vi "Offset Measurement Next Phase.vi"(6 "zero":T1, 8 "error in (no error)":errorcluster, 9 "Status":T4=enum."created", 10 "Offset Measurement":T2={"phase"=enum."idle", "measureInputOffset"={"buffers"=0, "settle"=2, "timeout"=5.0, "channels"=[], "zero"=enum."both"}, "settle remaining"=0, "buffers remaining"=0, "deadline"=0, "sum"=[], "count"=0, "saved amplitudes"=[], "saved offsets"=[], "previous status"=enum."created"}, 11 "Instrument.DAQ in":refnum<class "Instrument.DAQ.lvclass">) -> (0 "error out":errorcluster, 2 "Offset Measurement":T2={"phase"=enum."idle", "measureInputOffset"={"buffers"=0, "settle"=2, "timeout"=5.0, "channels"=[], "zero"=enum."both"}, "settle remaining"=0, "buffers remaining"=0, "deadline"=0, "sum"=[], "count"=0, "saved amplitudes"=[], "saved offsets"=[], "previous status"=enum."created"}, 3 "Instrument.DAQ out":refnum<class "Instrument.DAQ.lvclass">)   [LabVIEW 2019, in "Instrument.Lockin.lvlib" / "Instrument.DAQ.lvclass"]
uses:
  Instrument.DAQ.lvclass
  Typedefs/Offset Measurement--Cluster.ctl
  Lockin.Typedefs/API/Lockin.measureInputOffset Config--Cluster.ctl
  Lockin.Typedefs/API/Lockin.measureInputOffset.zero--enum.ctl
  Lockin.Typedefs/other/Status--enum.ctl
  Instrument.DAQ.lvclass/Instrument.DAQ.ctl
  Lockin.Typedefs/Lockin.Typedefs.lvlib
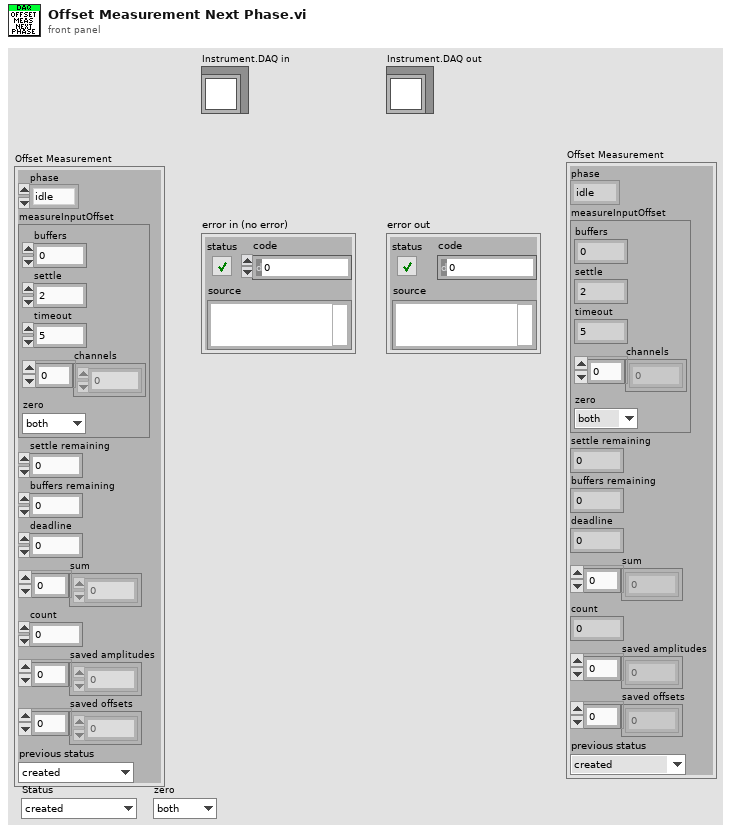
[diagram p1: front panel]
types:
  T1 = typedef "Lockin.Typedefs.lvlib/Lockin.measureInputOffset.zero--enum.ctl" = enum16{"both", "ac", "dc", "none"}
  T2 = typedef "Instrument.Lockin.lvlib/Instrument.DAQ.lvclass/Offset Measurement--Cluster.ctl" = cluster{"phase":enum16{"idle", "zeroing", "settling", "averaging", "done", "aborted", "cancelled", "timed out"}, "measureInputOffset":T3, "settle remaining":i32, "buffers remaining":i32, "deadline":u32, "sum":dbl[], "count":i32, "saved amplitudes":dbl[], "saved offsets":dbl[], "previous status":T4}
  T3 = typedef "Lockin.Typedefs.lvlib/Lockin.measureInputOffset Config--Cluster.ctl" = cluster{"buffers":i32, "settle":i32, "timeout":dbl, "channels":i32[], "zero":T1}
  T4 = typedef "Lockin.Typedefs.lvlib/Status--enum.ctl" = enum16{"idle", "created", "started", "stopped", "sweeping", "measuring offset"}
  T5 = enum16{"idle", "zeroing", "settling", "averaging", "done", "aborted", "cancelled", "timed out"}
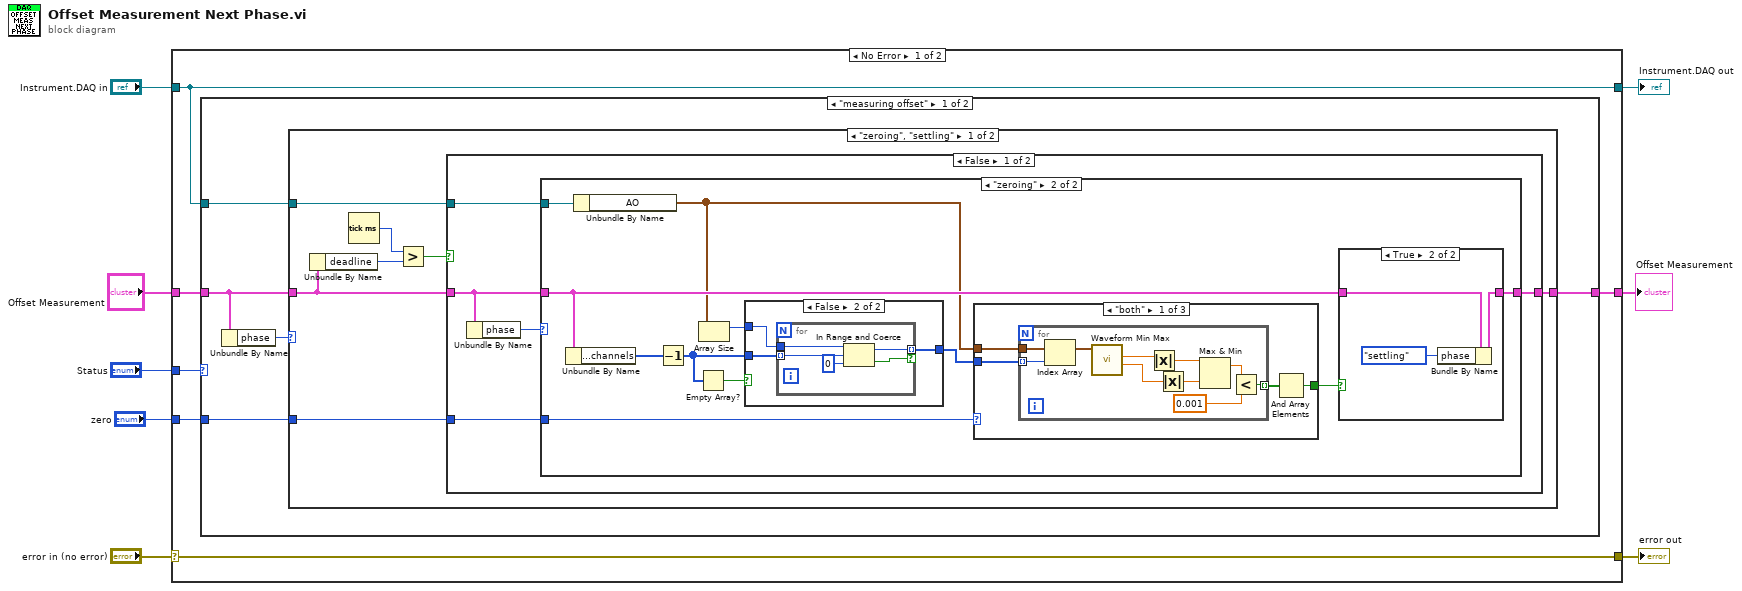
[diagram p0: block diagram]
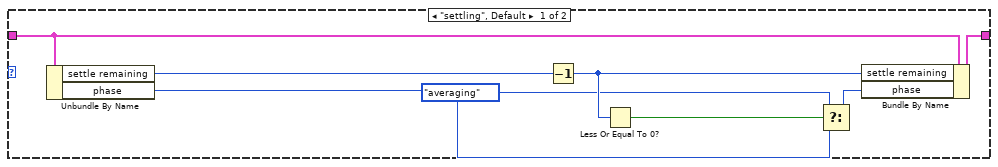
[diagram p2: hidden frame]
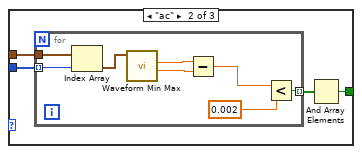
[diagram p4: hidden frame]
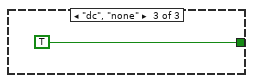
[diagram p5: hidden frame]
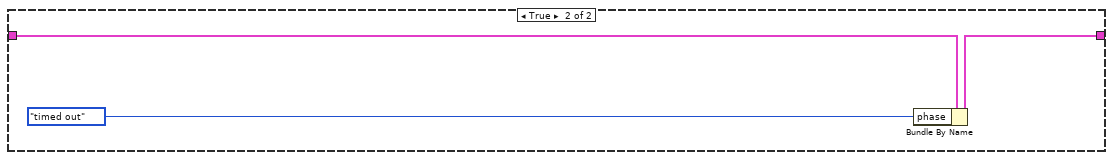
[diagram p7: hidden frame]
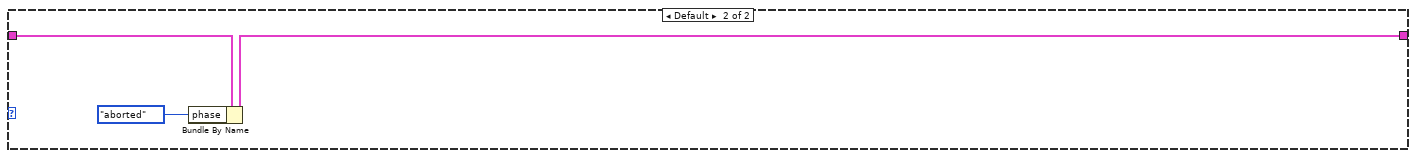
[diagram p9: hidden frame]
diagram:
  n1 = case shown="No Error" "error in (no error)" {
    selector: "error in (no error)" -> [w10 w102]
    tunnel: "Offset Measurement" -> [w14 w100]
    tunnel: [w13 w100] -> w7
    tunnel: "Status" -> [w12 _]
    tunnel: "Instrument.DAQ in" -> [w11 w101]
    tunnel: [w11 w101] -> w3
    tunnel: [w10 w102] -> w2
    tunnel: "zero" -> [w9 _]
    frame No Error {
      n2 = case shown="\"measuring offset\"" w12 {
        tunnel: w14 -> [w19 w99]
        tunnel: [w18 w97] -> w13
        tunnel: w11 -> [w17 _]
        tunnel: w9 -> [w15 _]
        frame "measuring offset" {
          n3 = Unbundle By Name(w19) -> ("phase"=w16:T5)
          n4 = case shown="\"zeroing\", \"settling\"" w16 {
            tunnel: w19 -> [w24 w96]
            tunnel: [w22 w96] -> w18
            tunnel: w17 -> [w21 _]
            tunnel: w15 -> [w20 _]
            frame "zeroing", "settling" {
              n5 = Unbundle By Name(w24) -> ("deadline"=w26:u32)
              n6 = Tick Count (ms)() -> (millisecond timer value=w25:u32)
              n7 = Greater?(x=w25, y=w26) -> (0:w23:bool)
              n8 = case shown="False" w23 {
                tunnel: w24 -> [w30 w95]
                tunnel: [w29 w93] -> w22
                tunnel: w21 -> [w28 _]
                tunnel: w20 -> [w27 _]
                frame False {
                  n9 = Unbundle By Name(w30) -> ("phase"=w31:T5)
                  n10 = case shown="\"zeroing\"" w31 {
                    tunnel: w30 -> [w38 w46]
                    tunnel: [w37 w50] -> w29
                    tunnel: w28 -> [_ w49]
                    tunnel: w27 -> [_ w47]
                    frame "settling", Default {
                      n11 = Unbundle By Name(w38) -> ("settle remaining"=w39:i32, "phase"=w32:T5)
                      n12 = Decrement(x=w39) -> (x-1=w36:i32)
                      n13 = Less Or Equal To 0?(x=w36) -> (x <= 0?=w33:bool)
                      n14 = Select(t=T5."averaging" ("phase"), s=w33, f=w32) -> (s? t:f=w34:T5)
                      n15 = Bundle By Name(cluster=w38, "settle remaining"=w36, "phase"=w34) -> (w37:T2)
                    }
                    frame "zeroing" {
                      n16 = Unbundle By Name(w46) -> ("measureInputOffset.channels"=w45:i32[])
                      n17 = Unbundle By Name(w49) -> ("AO"=w42:waveform(dbl)[])
                      n18 = Decrement(x=w45) -> (x-1=w43:i32[])
                      n19 = Empty Array?(array=w43) -> (empty?=w44:bool)
                      n20 = Array Size(array=w42) -> (size(s)=w41:i32)
                      n21 = case shown="False" w44 {
                        tunnel: [w52 w56] -> w40
                        tunnel: w43 -> [_ w55]
                        tunnel: w41 -> [w51 w54]
                        frame True {
                          n22 = for {
                            N: w51 -> [_]
                            tunnel: [w53] -> w52 mode=indexing
                            i -> [w53]
                          }
                        }
                        frame False {
                          n23 = for {
                            tunnel: [w58] -> w56 mode=indexing if=w57
                            tunnel: w55 -> [w61] mode=indexing
                            tunnel: w54 -> [w59]
                            n24 = In Range and Coerce(upper limit=w59, x=w61, lower limit=0) -> (coerced(x)=w58:i32, In Range?=w57:bool)
                          }
                        }
                      }
                      n25 = case shown="\"both\"" w47 {
                        tunnel: w42 -> [w63 w77 _]
                        tunnel: [w65 w79 TRUE] -> w48
                        tunnel: w40 -> [w62 w76 _]
                        frame "both" {
                          n26 = for {
                            tunnel: [w69] -> w64 mode=indexing
                            tunnel: w63 -> [w68]
                            tunnel: w62 -> [w66] mode=indexing
                            n27 = Index Array(array=w68, index=w66) -> (element=w67:waveform(dbl))
                            n28 = call <vilib>:"Waveform Min Max.vi"("waveform in"=w67) -> ("Y min"=w74:dbl, "Y max"=w75:dbl)  [unwired: 5 in, 4 out]
                            n29 = Absolute Value(x=w75) -> (abs(x)=w72:dbl)
                            n30 = Absolute Value(x=w74) -> (abs(x)=w73:dbl)
                            n31 = Max & Min(x=w72, y=w73) -> (max(x,y)=w71:dbl)  [unwired: 1 out]
                            n32 = Less?(x=w71, y=0.001) -> (x < y?=w69:bool)
                          }
                          n33 = And Array Elements(Boolean array=w64) -> (logical AND=w65:bool)
                        }
                        frame "ac" {
                          n34 = for {
                            tunnel: [w86] -> w78 mode=indexing
                            tunnel: w77 -> [w82]
                            tunnel: w76 -> [w80] mode=indexing
                            n35 = Index Array(array=w82, index=w80) -> (element=w81:waveform(dbl))
                            n36 = call <vilib>:"Waveform Min Max.vi"("waveform in"=w81) -> ("Y min"=w84:dbl, "Y max"=w85:dbl)  [unwired: 5 in, 4 out]
                            n37 = Subtract(x=w85, y=w84) -> (x-y=w83:dbl)
                            n38 = Less?(x=w83, y=0.002) -> (x < y?=w86:bool)
                          }
                          n39 = And Array Elements(Boolean array=w78) -> (logical AND=w79:bool)
                        }
                        frame "dc", "none" {
                        }
                      }
                      n40 = case shown="True" w48 {
                        tunnel: w46 -> [w89 w91]
                        tunnel: [w89 w90] -> w50
                        frame False {
                        }
                        frame True {
                          n41 = Bundle By Name(cluster=w91, "phase"=T5."settling") -> (w90:T2)
                        }
                      }
                    }
                  }
                }
                frame True {
                  n42 = Bundle By Name(cluster=w95, "phase"=T5."timed out") -> (w93:T2)
                }
              }
            }
            frame Default {
            }
          }
        }
        frame Default {
          n43 = Bundle By Name(cluster=w99, "phase"=T5."aborted") -> (w97:T2)
        }
      }
    }
    frame Error {
    }
  }
  "error out" <- w2
  "Instrument.DAQ out" <- w3
  "Offset Measurement" <- w7
